vi "Sous_VI_Monter_Bras.vi"(8 "error in (no error)":errorcluster) -> (0 "error out":errorcluster)   [LabVIEW 2017]
uses:
  enum_bras.ctl
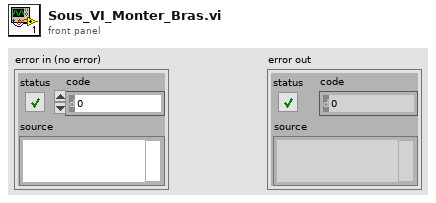
[diagram p1: front panel]
types:
  T1 = typedef "enum_bras.ctl" = enum16{"Depart Bras", "Clapet Bras", "Inactif Bras", "Seaux Bras"}
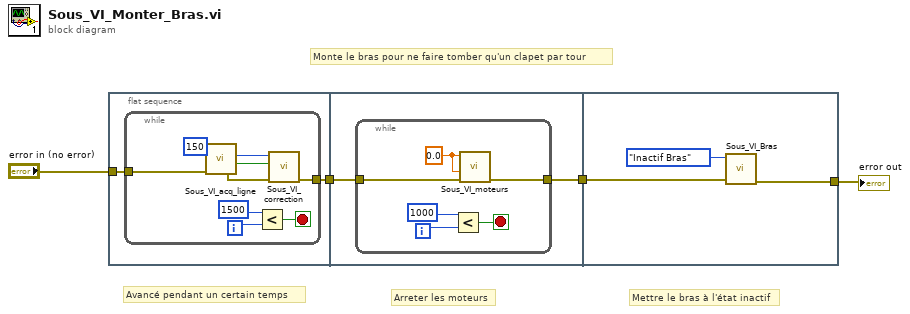
[diagram p0: block diagram]
diagram:
  # "Mettre le bras à l'état inactif"
  # "Arreter les moteurs"
  # "Avancé pendant un certain temps"
  # "Monte le bras pour ne faire tomber qu'un clapet par tour"
  n1 = flat-sequence {
    tunnel: "error in (no error)" -> [w6]
    tunnel: [w5] -> w2
    tunnel: w2 -> [w17]
    tunnel: [w16] -> w1
    tunnel: [w25] -> w4
    tunnel: w1 -> [w24]
    frame #0 {
      n2 = while {
        tunnel: w6 -> [w10]
        tunnel: [w7] -> w5
        i -> [w15]
        stop <- w13 stop-if-true
        n3 = call "Sous_VI_acq_ligne.vi"("Seuil"=150, "error in (no error)"=w10) -> ("Décalage"=w12:u32, "G/D ?"=w9:bool, "error out"=w8:errorcluster)  [unwired: 8 in, 3 out]
        n4 = Less?(x=1500, y=w15) -> (x < y?=w13:bool)
        n5 = call "Sous_VI_correction.vi"("error in (no error)"=w8, "G/D ?"=w9, "Décalage"=w12) -> ("error out"=w7:errorcluster)  [unwired: 8 in]
      }
    }
    frame #1 {
      n6 = while {
        tunnel: w17 -> [w19]
        tunnel: [w18] -> w16
        i -> [w23]
        stop <- w21 stop-if-true
        w20 = 0.0 ("moteur gauche vite")
        n7 = Less?(x=1000, y=w23) -> (x < y?=w21:bool)
        n8 = call "Sous_VI_moteurs.vi"("error in (no error)"=w19, "Moteur Droit"=w20, "Moteur Gauche"=w20) -> ("error out"=w18:errorcluster)  [unwired: 8 in]
      }
    }
    frame #2 {
      n9 = call "Sous_VI_Bras.vi"("error in (no error)"=w24, "Enum bras"=enum_bras."Inactif Bras") -> ("error out"=w25:errorcluster)  [unwired: 9 in]
    }
  }
  "error out" <- w4
